vi "Disable Logger by Name.vi"(8 "error in (no error)":errorcluster, 11 "name (\"Default\")":string="Default") -> (0 "error out":errorcluster)   [LabVIEW 2018, in "GLog.lvlib"]
doc: "Disables a specific logger in the Registry by name.\n\nIf the name provided does not match any currently registered loggers, this VI will return an error."
uses:
  GLog.lvlib
  registry/Registry.lvlib
panel:
  # "Connector Pane"
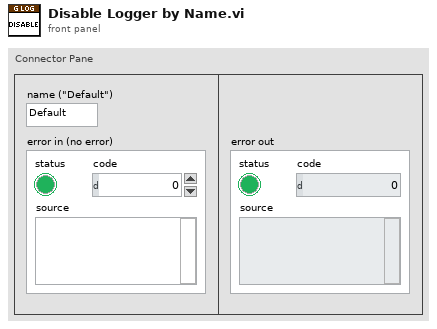
[diagram p1: front panel]
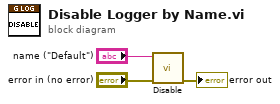
[diagram p0: block diagram]
diagram:
  n1 = call "Disable.vi"("error in (no error)"="error in (no error)", "logger name"="name (\"Default\")") -> ("error out"=→"error out":errorcluster)  [unwired: 9 in]
